vi "Update Listbox headers.vi"(7 "Interpret as Unicode (T)":bool=TRUE, 8 "error in (no error)":errorcluster, 10 "Column Header":string, 11 "Listbox Ref":refnum<vi>) -> (0 "error out":errorcluster, 3 "Listbox Ref":refnum<vi>)   [LabVIEW 2019, in "Language Selection.lvlib"]
doc: "Uses \"Column Header\" input string to translate a headers of a Listbox control.\n- - -\nCopyright (c) 2026, Merecs Engineering GmbH"
uses:
  Language Selection.lvlib
panel:
  # "Connector Pane"
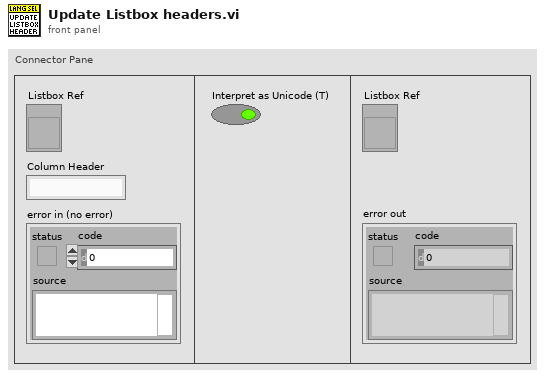
[diagram p1: front panel]
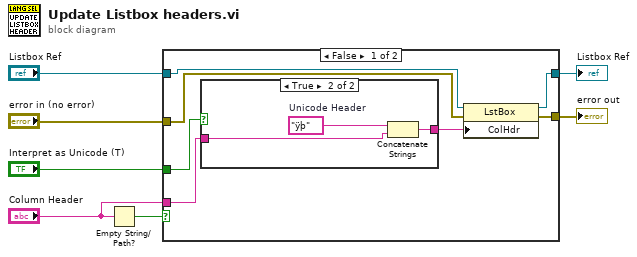
[diagram p0: block diagram]
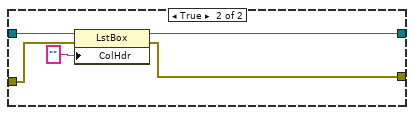
[diagram p3: hidden frame]
diagram:
  n1 = Empty String/Path?(string/path="Column Header") -> (empty?=w1:bool)
  n2 = case shown="False" w1 {
    tunnel: "Column Header" -> [w14 _]
    tunnel: [w13 w22] -> w5
    tunnel: "error in (no error)" -> [w12 w21]
    tunnel: "Listbox Ref" -> [w11 w20]
    tunnel: "Interpret as Unicode (T)" -> [w10 _]
    tunnel: [w9 w23] -> w6
    frame False {
      n3 = case shown="True" w10 {
        tunnel: w14 -> [w15 w18]
        tunnel: [w15 w17] -> w8
        frame False {
        }
        frame True {
          w16 = "ÿþ"  # Unicode Header
          n4 = Concatenate Strings(w16, w18) -> (w17:string)
        }
      }
      n5 = property class="LstBox"(reference=w11, error in=w12, "ColHdr"=w8) -> (reference out=w9:refnum<vi>, error out=w13:errorcluster)
    }
    frame True {
      n6 = property class="LstBox"(reference=w20, error in=w21, "ColHdr"="") -> (reference out=w23:refnum<vi>, error out=w22:errorcluster)
    }
  }
  "error out" <- w5
  "Listbox Ref" <- w6
